vi "Cluster Ops Probe.vi"() -> ()   [LabVIEW 2026]
doc: "Round6 Task3 probe: cluster operation node coverage in AIXML. Bundle uses the append-only idiom: a TYPED EMPTY cluster constant (value=\"\") as the cluster: base plus element: inputs. Expected: Bundle Out={1,two,3.5}, Unbundled A=1, Unbundled B=two, Unbundled C=3.5, ByName A=1, ByName C=3.5, BundleByName Out={1,TWO-REPLACED,3.5}."
panel:
  out "ByName C":dbl
  out "ByName A":i32
  out "BundleByName Out":T1={"Field A"=0, "Field B"="\"\"", "Field C"=0.0}
  out "Unbundled C":dbl
  out "Unbundled B":string
  out "Unbundled A":i32
  out "Bundle Out":cluster{i32, string, dbl}={0, "\"\"", 0.0}
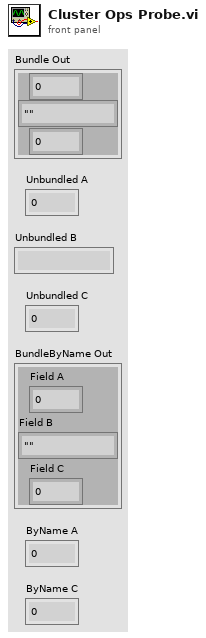
[diagram p1: front panel]
types:
  T1 = cluster{"Field A":i32, "Field B":string, "Field C":dbl}
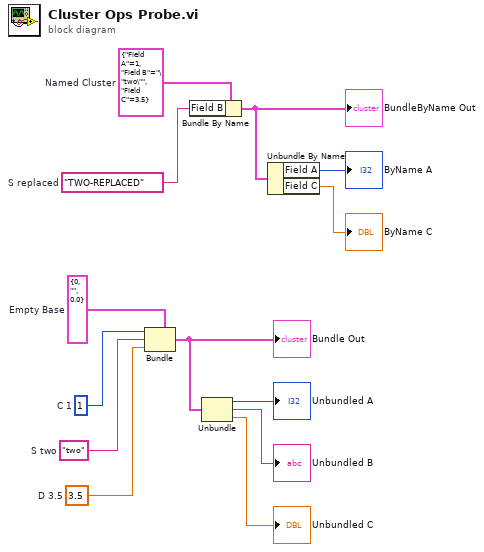
[diagram p0: block diagram]
diagram:
  w8 = T1 {"Field A"=1, "Field B"="\"two\"", "Field C"=3.5}  # Named Cluster
  w13 = cluster{i32, string, dbl} {0, "", 0.0}  # Empty Base
  w9 = "TWO-REPLACED"  # S replaced
  w10 = 3.5  # D 3.5
  w11 = "two"  # S two
  w12 = 1  # C 1
  n1 = Bundle(cluster=w13, w12, w11, w10) -> (w7:cluster{i32, string, dbl})
  "Bundle Out" <- w7
  n2 = Bundle By Name(cluster=w8, "Field B"=w9) -> (w3:T1)
  "BundleByName Out" <- w3
  n3 = Unbundle(w7) -> (→"Unbundled A":i32, →"Unbundled B":string, →"Unbundled C":dbl)
  n4 = Unbundle By Name(w3) -> ("Field A"=→"ByName A":i32, "Field C"=→"ByName C":dbl)
